vi "SeqEditor_updateData.vi"(8 "error in (no error)":errorcluster, 11 "NLTest in":refnum<class "NLTest.lvclass">) -> (0 "error out":errorcluster, 3 "NLTest out":refnum<class "NLTest.lvclass">)   [LabVIEW 2017, in "NLTest.lvclass"]
uses:
  NLTest.lvclass
  NLTest.lvclass/NLTest.ctl
panel:
  # "反向更新\n1、更新到总数据\n2、依据列2数据，更新列0，1"
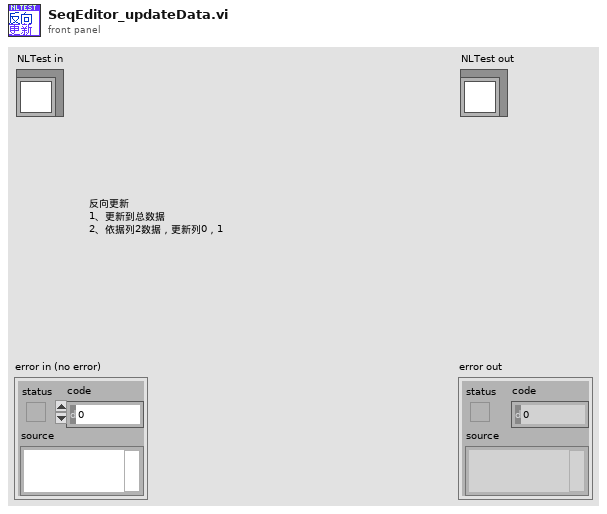
[diagram p1: front panel]
types:
  T1 = typedef "NLTest.lvclass/allseqanddata.ctl" = cluster{"seqname":string, "seqdata":string[]}
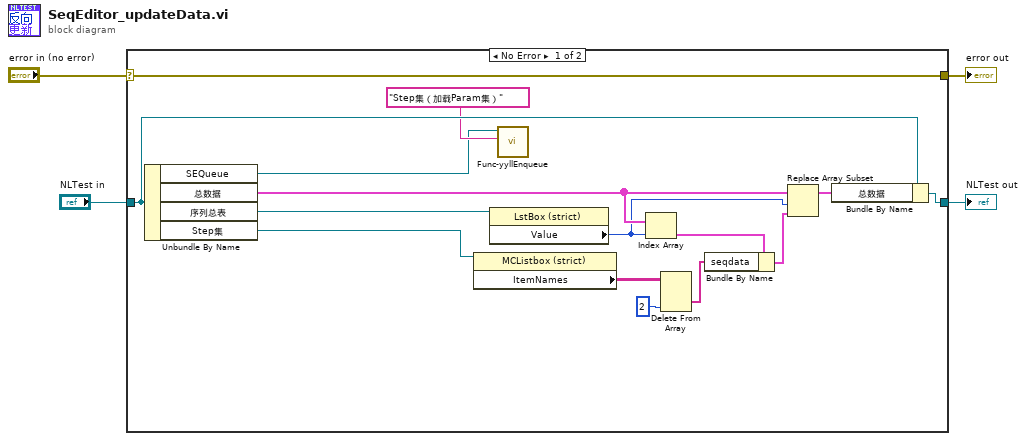
[diagram p0: block diagram]
diagram:
  n1 = case shown="No Error" "error in (no error)" {
    selector: "error in (no error)" -> [w19 w21]
    tunnel: [w19 w21] -> w3
    tunnel: [w10 w20] -> w1
    tunnel: "NLTest in" -> [w18 w20]
    frame No Error {
      n2 = Unbundle By Name(w18) -> ("SEQueue"=w5:refnum<queue>, "总数据"=w15:T1[], "序列总表"=w17:refnum<vi>, "Step集"=w16:refnum<vi>)
      n3 = property class="MCListbox (strict)"(reference=w16) -> ("ItemNames"=w13:string[][])  [unwired: 1 in, 2 out]
      n4 = property class="LstBox (strict)"(reference=w17) -> ("Value"=w14:i32)  [unwired: 1 in, 2 out]
      n5 = call "Func-yyllEnqueue.vi"("cmd"="Step集（加载Param集）", "queue in"=w5) -> ()  [unwired: 7 in, 3 out]
      n6 = Index Array(array=w15, index=w14) -> (element=w8:T1)
      n7 = Delete From Array(array=w13, index (col)=2 ("disabled index (col)")) -> (deleted portion=w11:string[])  [unwired: 2 in, 1 out]
      n8 = Bundle By Name(cluster=w8, "seqdata"=w11) -> (w7:T1)
      n9 = Replace Array Subset(array=w15, new element=w7, index=w14) -> (w9:T1[])
      n10 = Bundle By Name(cluster=w18, "总数据"=w9) -> (w10:refnum<class "NLTest.lvclass">)
    }
    frame Error {
    }
  }
  "error out" <- w3
  "NLTest out" <- w1
